vi "DrawSubMenu.vi"(7 "Tag":string, 8 "error in (no error)":errorcluster, 9 "Pict Refnum":refnum<vi>, 10 "Coords":T2, 11 "Menu in":refnum<class "Menu.lvclass">) -> (0 "error out":errorcluster, 1 "Global Area":T1, 2 "Selected Area":T1, 3 "Menu out":refnum<class "Menu.lvclass">, 4 "SubMenu":bool, 5 "Selected Tag":string)   [LabVIEW 2021, in "Menu.lvlib" / "Menu.lvclass"]
uses:
  Menu.lvclass
  <vilib>/Utility/miscctls.llb/LVPoint32TypeDef.ctl
  Picture2D/src/Collection/Collection.lvclass
  C:/GitHub/Picture2D/src/IDrawable/IDrawable.lvclass
  Picture2D/src/2DPictureControl/2DPictureControl.lvclass
  Picture2D/src/PointSpecialized/PointSpecialized.lvclass
  C:/GitHub/Picture2D/src/Point/Point.lvclass
  Picture2D/src/Rectangle/Rectangle.lvclass
  C:/GitHub/Picture2D/src/Shape/Shape.lvclass
  C:/GitHub/Picture2D/src/Polygone/Polygone.lvclass
  <vilib>/picture/PictureSupport.llb/RectSize.vi
  GetMenuColors.vi
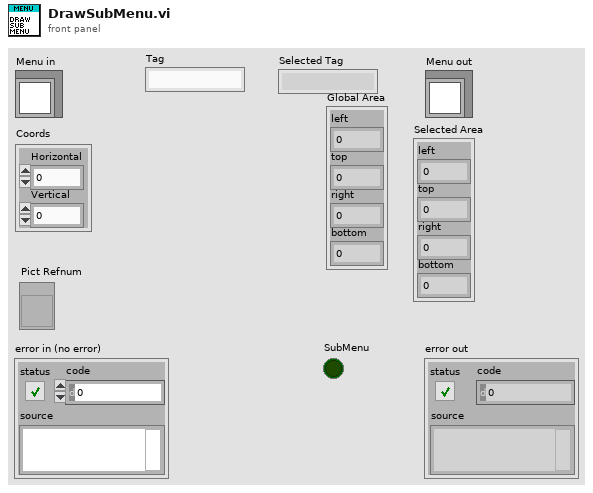
[diagram p1: front panel]
types:
  T1 = cluster{"left":i16, "top":i16, "right":i16, "bottom":i16}
  T2 = typedef "LVPoint32TypeDef.ctl" = cluster{"Horizontal":i32, "Vertical":i32}
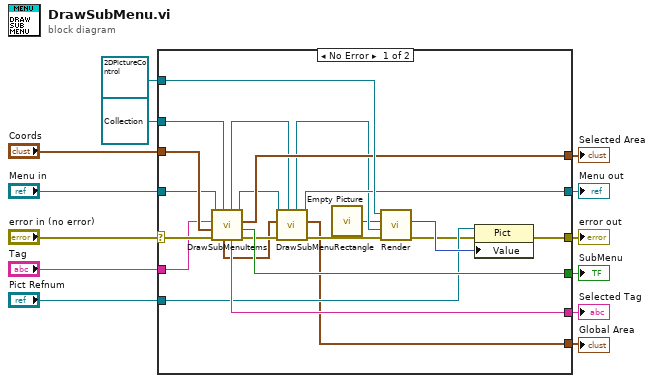
[diagram p0: block diagram]
diagram:
  n1 = case shown="No Error" "error in (no error)" {
    selector: "error in (no error)" -> [w28 w36]
    tunnel: [w34 _] -> w13
    tunnel: [w22 _] -> w12
    tunnel: [w33 w36] -> w11
    tunnel: [w32 _] -> w10
    tunnel: "Coords" -> [w30 _]
    tunnel: [w19 w37] -> w7
    tunnel: "Menu in" -> [w26 w37]
    tunnel: refnum<class "Collection.lvclass"> refnum ("Picture2D.lvlib:Collection.lvclass") -> [w27 _]
    tunnel: refnum<class "2DPictureControl.lvclass"> refnum ("2DPictureControl in") -> [w29 _]
    tunnel: "Pict Refnum" -> [w25 _]
    tunnel: "Tag" -> [w23 _]
    tunnel: [w17 _] -> w1
    frame No Error {
      n2 = call "DrawSubMenuItems.vi"("Collection in"=w27, "error in (no error)"=w28, "Coords"=w30, "Tag"=w23, "Menu in"=w26) -> ("error out"=w31:errorcluster, "SubMenu"=w32:bool, "SelectedArea"=w22:T1, "Menu out"=w20:refnum<class "Menu.lvclass">, "SelectedItemTag"=w34:string, "Collection out"=w16:refnum<class "Collection.lvclass">, "GlobalArea"=w18:T1)
      n3 = call "DrawSubMenuRectangle.vi"("Collection in"=w16, "error in (no error)"=w31, "Area"=w18, "Menu in"=w20) -> ("error out"=w21:errorcluster, "Area"=w17:T1, "Menu out"=w19:refnum<class "Menu.lvclass">, "Collection out"=w15:refnum<class "Collection.lvclass">)  [unwired: 4 in]
      n4 = call "Empty Picture"() -> ("empty picture"=w14:picture)
      n5 = call-dynamic "Render.vi"("error in (no error)"=w21, "IDrawable"=w15, "2D Picture in"=w14, "2DPictureControl in"=w29) -> ("error out"=w24:errorcluster, "2D Picture out"=w35:picture)  [unwired: 5 in, 1 out]
      n6 = property class="Pict"(reference=w25, error in=w24, "Value"=w35) -> (error out=w33:errorcluster)  [unwired: 1 out]
    }
    frame Error {
    }
  }
  "Selected Tag" <- w13
  "Selected Area" <- w12
  "error out" <- w11
  "Menu out" <- w7
  "SubMenu" <- w10
  "Global Area" <- w1
